vi "Current_Setting_1_7_26.vi"() -> ()   [LabVIEW 2025]
uses:
  <vilib>/addons/zeromq/zmq_socket.lvclass
  <vilib>/Waveform/DWDTOps.llb/DWDT Digital to Boolean Array.vi
  GV_TC1_M.vi
  <vilib>/DAQmx/read.llb/DAQmx Read (Analog DBL 1Chan 1Samp).vi
  <vilib>/DAQmx/read.llb/DAQmx Read (Analog 1D DBL NChan 1Samp).vi
  GV_TC1.vi
  <vilib>/addons/zeromq/zmq_context.lvclass
  <vilib>/addons/zeromq/socket_type.ctl
  <vilib>/addons/zeromq/zeromq.lvlib
  <vilib>/DAQmx/create/channels.llb/DAQmx Create Channel (AI-Voltage-Basic).vi
  <resource>/objmgr/daqmx.rc
  <vilib>/DAQmx/create/channels.llb/DAQmx Create Channel (AO-Voltage-Basic).vi
  <vilib>/DAQmx/write.llb/DAQmx Write (Analog DBL 1Chan 1Samp).vi
  GV_TC9_Mo.vi
panel:
  in  "stop":bool
  out "TC1_Command":dbl
  out "Waveform Chart":dbl(graph)
  out "Sign*10":dbl
  in  "Error_TC9":dbl
  in  "Inc/Dec":dbl
  in  "RF":tag
  in  "Others":tag
  out "error out":errorcluster
  out "double precision float":dbl
  out "Source 1":dbl
  out "Source 2":dbl
  out "Source 3":dbl
  out "Source 4":dbl
  out "Source 5":dbl
  out "Source 6":dbl
  out "Source 7":dbl
  out "Source 8":dbl
  out "Source 9":dbl
  out "Source 10":dbl
  out "Source 11":dbl
  out "Source 12":dbl
  out "Source 13":dbl
  out "Source 14":dbl
  out "value":dbl[](array[numeric])
  out "subarray":dbl[](array[numeric])
  out "Boolean array":bool[](array[boolean])
  out "TC 1":dbl
  out "TC 2":dbl
  out "TC 3":dbl
  out "TC 4":dbl
  out "TC 5":dbl
  out "TC 6":dbl
  out "TC 7":dbl
  out "TC 8":dbl
  out "going to Device 9":dbl
  out "going to Device 10":dbl
  out "going to Device 11":dbl
  out "going to Device 12":dbl
  out "going to Device 13":dbl
  out "going to Device 14":dbl
  in  "Numerator":dbl
  in  "Denominator":dbl
  in  "Inc/Dec 2":dbl
  in  "Error_Stop":dbl
  in  "Boolean":bool
  out "Array":dbl[](array[numeric])
  out "max value":i16
  out "Array[0]":dbl
  out "max value 2":i16
  out "Array 2":dbl[](array[numeric])
  in  "TP1":dbl
  in  "TP2":dbl
  in  "RF 2":dbl
  in  "Beam":dbl
  in  "Boolean 2":bool
  in  "Boolean 3":bool
  out "[0]":bool
  out "[1]":bool
  out "[2]":bool
  out "[3]":bool
  out "others":dbl[](array[numeric]) format="%0.2f"
  out "appended array":dbl[](array[numeric])
  out "x/y":dbl
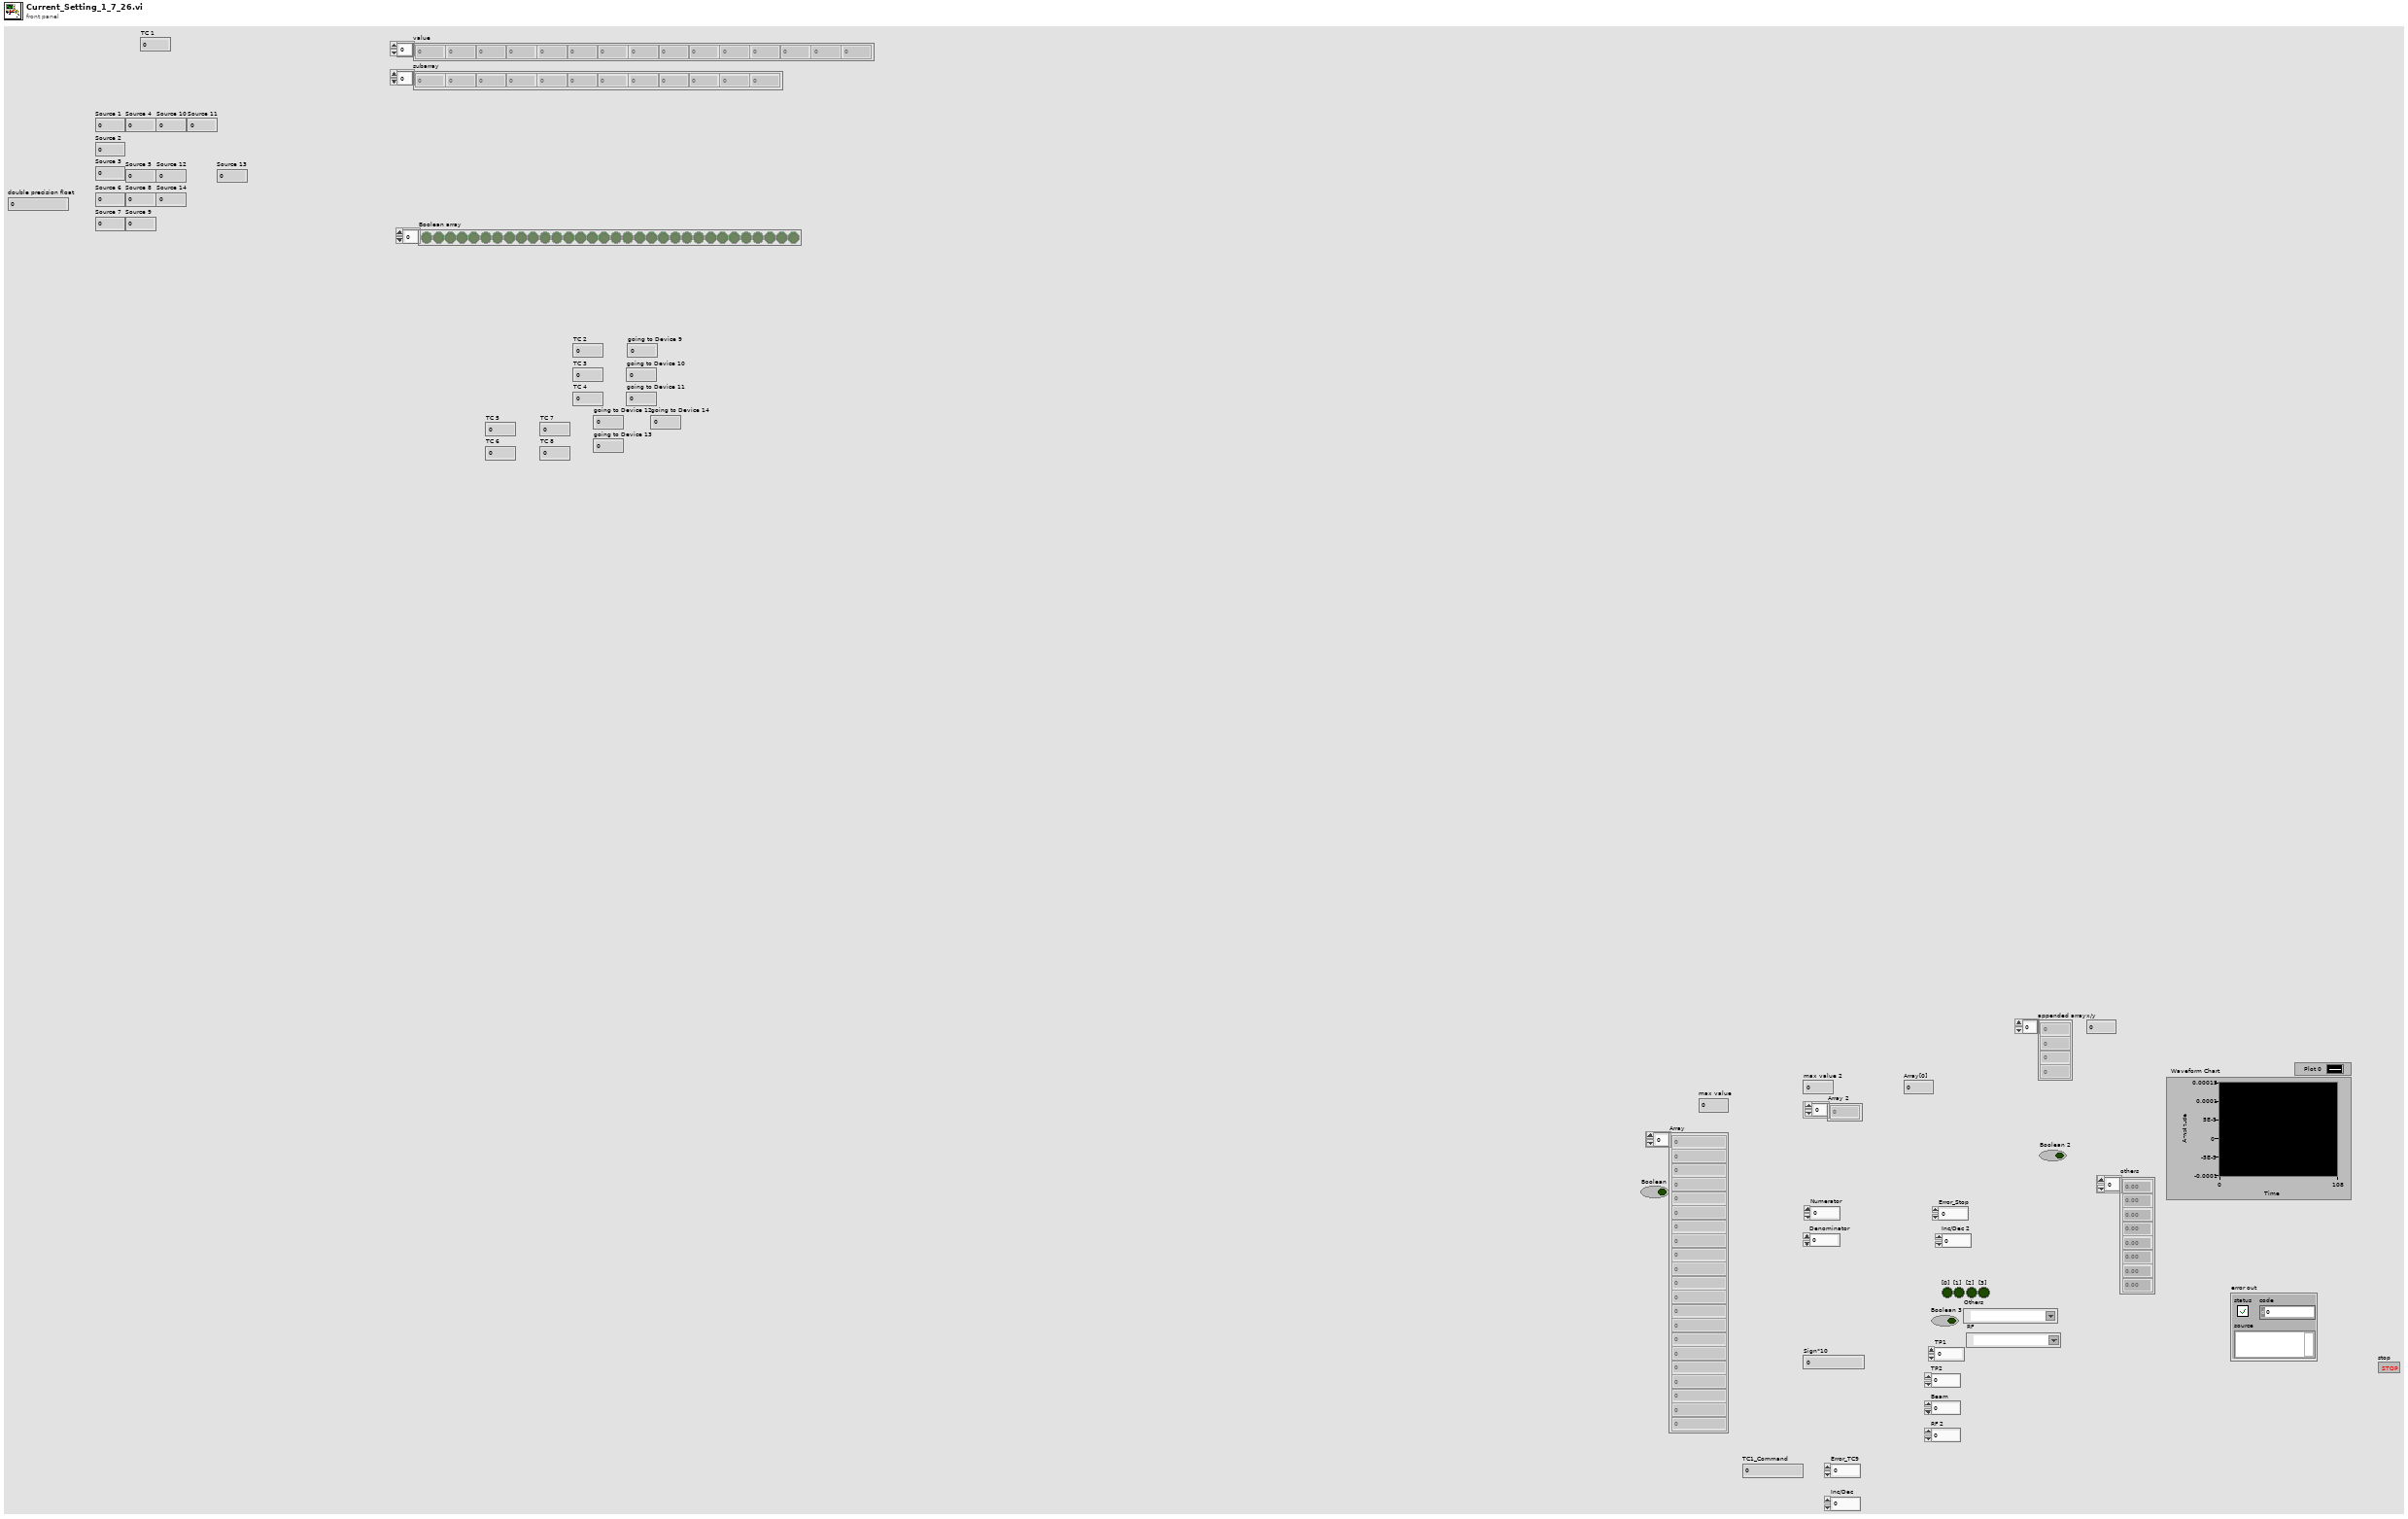
[diagram p1: front panel]
types:
  T1 = typedef "zeromq.lvlib/socket_type.ctl" = enum8{"ZMQ_PAIR", "ZMQ_PUB", "ZMQ_SUB", "ZMQ_REQ", "ZMQ_REP", "ZMQ_DEALER", "ZMQ_ROUTER", "ZMQ_PULL", "ZMQ_PUSH", "ZMQ_XPUB", "ZMQ_XSUB", "ZMQ_STREAM", "ZMQ_SERVER", "ZMQ_CLIENT", "ZMQ_RADIO", "ZMQ_DISH", "ZMQ_GATHER", "ZMQ_SCATTER", "ZMQ_DGRAM"}
  T2 = enum16{"big-endian, network order", "native, host order", "little-endian"}
  T3 = cluster{"[0]":bool, "[1]":bool, "[2]":bool, "[3]":bool, "[4]":bool, "[5]":bool, "[6]":bool, "[7]":bool, "[8]":bool}
  T4 = cluster{"[0]":dbl, "[1]":dbl, "[2]":dbl, "[3]":dbl, "[4]":dbl, "[5]":dbl, "[6]":dbl, "[7]":dbl}
  T5 = cluster{"Array[0]":dbl, "Array[1]":dbl, "Array[2]":dbl, "Array[3]":dbl, "Array[4]":dbl, "Array[5]":dbl, "Array[6]":dbl, "Array[7]":dbl}
  T6 = cluster{"[0]":digitalwaveform, "[1]":digitalwaveform, "[2]":digitalwaveform, "[3]":digitalwaveform, "[4]":digitalwaveform, "[5]":digitalwaveform, "[6]":digitalwaveform, "[7]":digitalwaveform, "[8]":digitalwaveform}
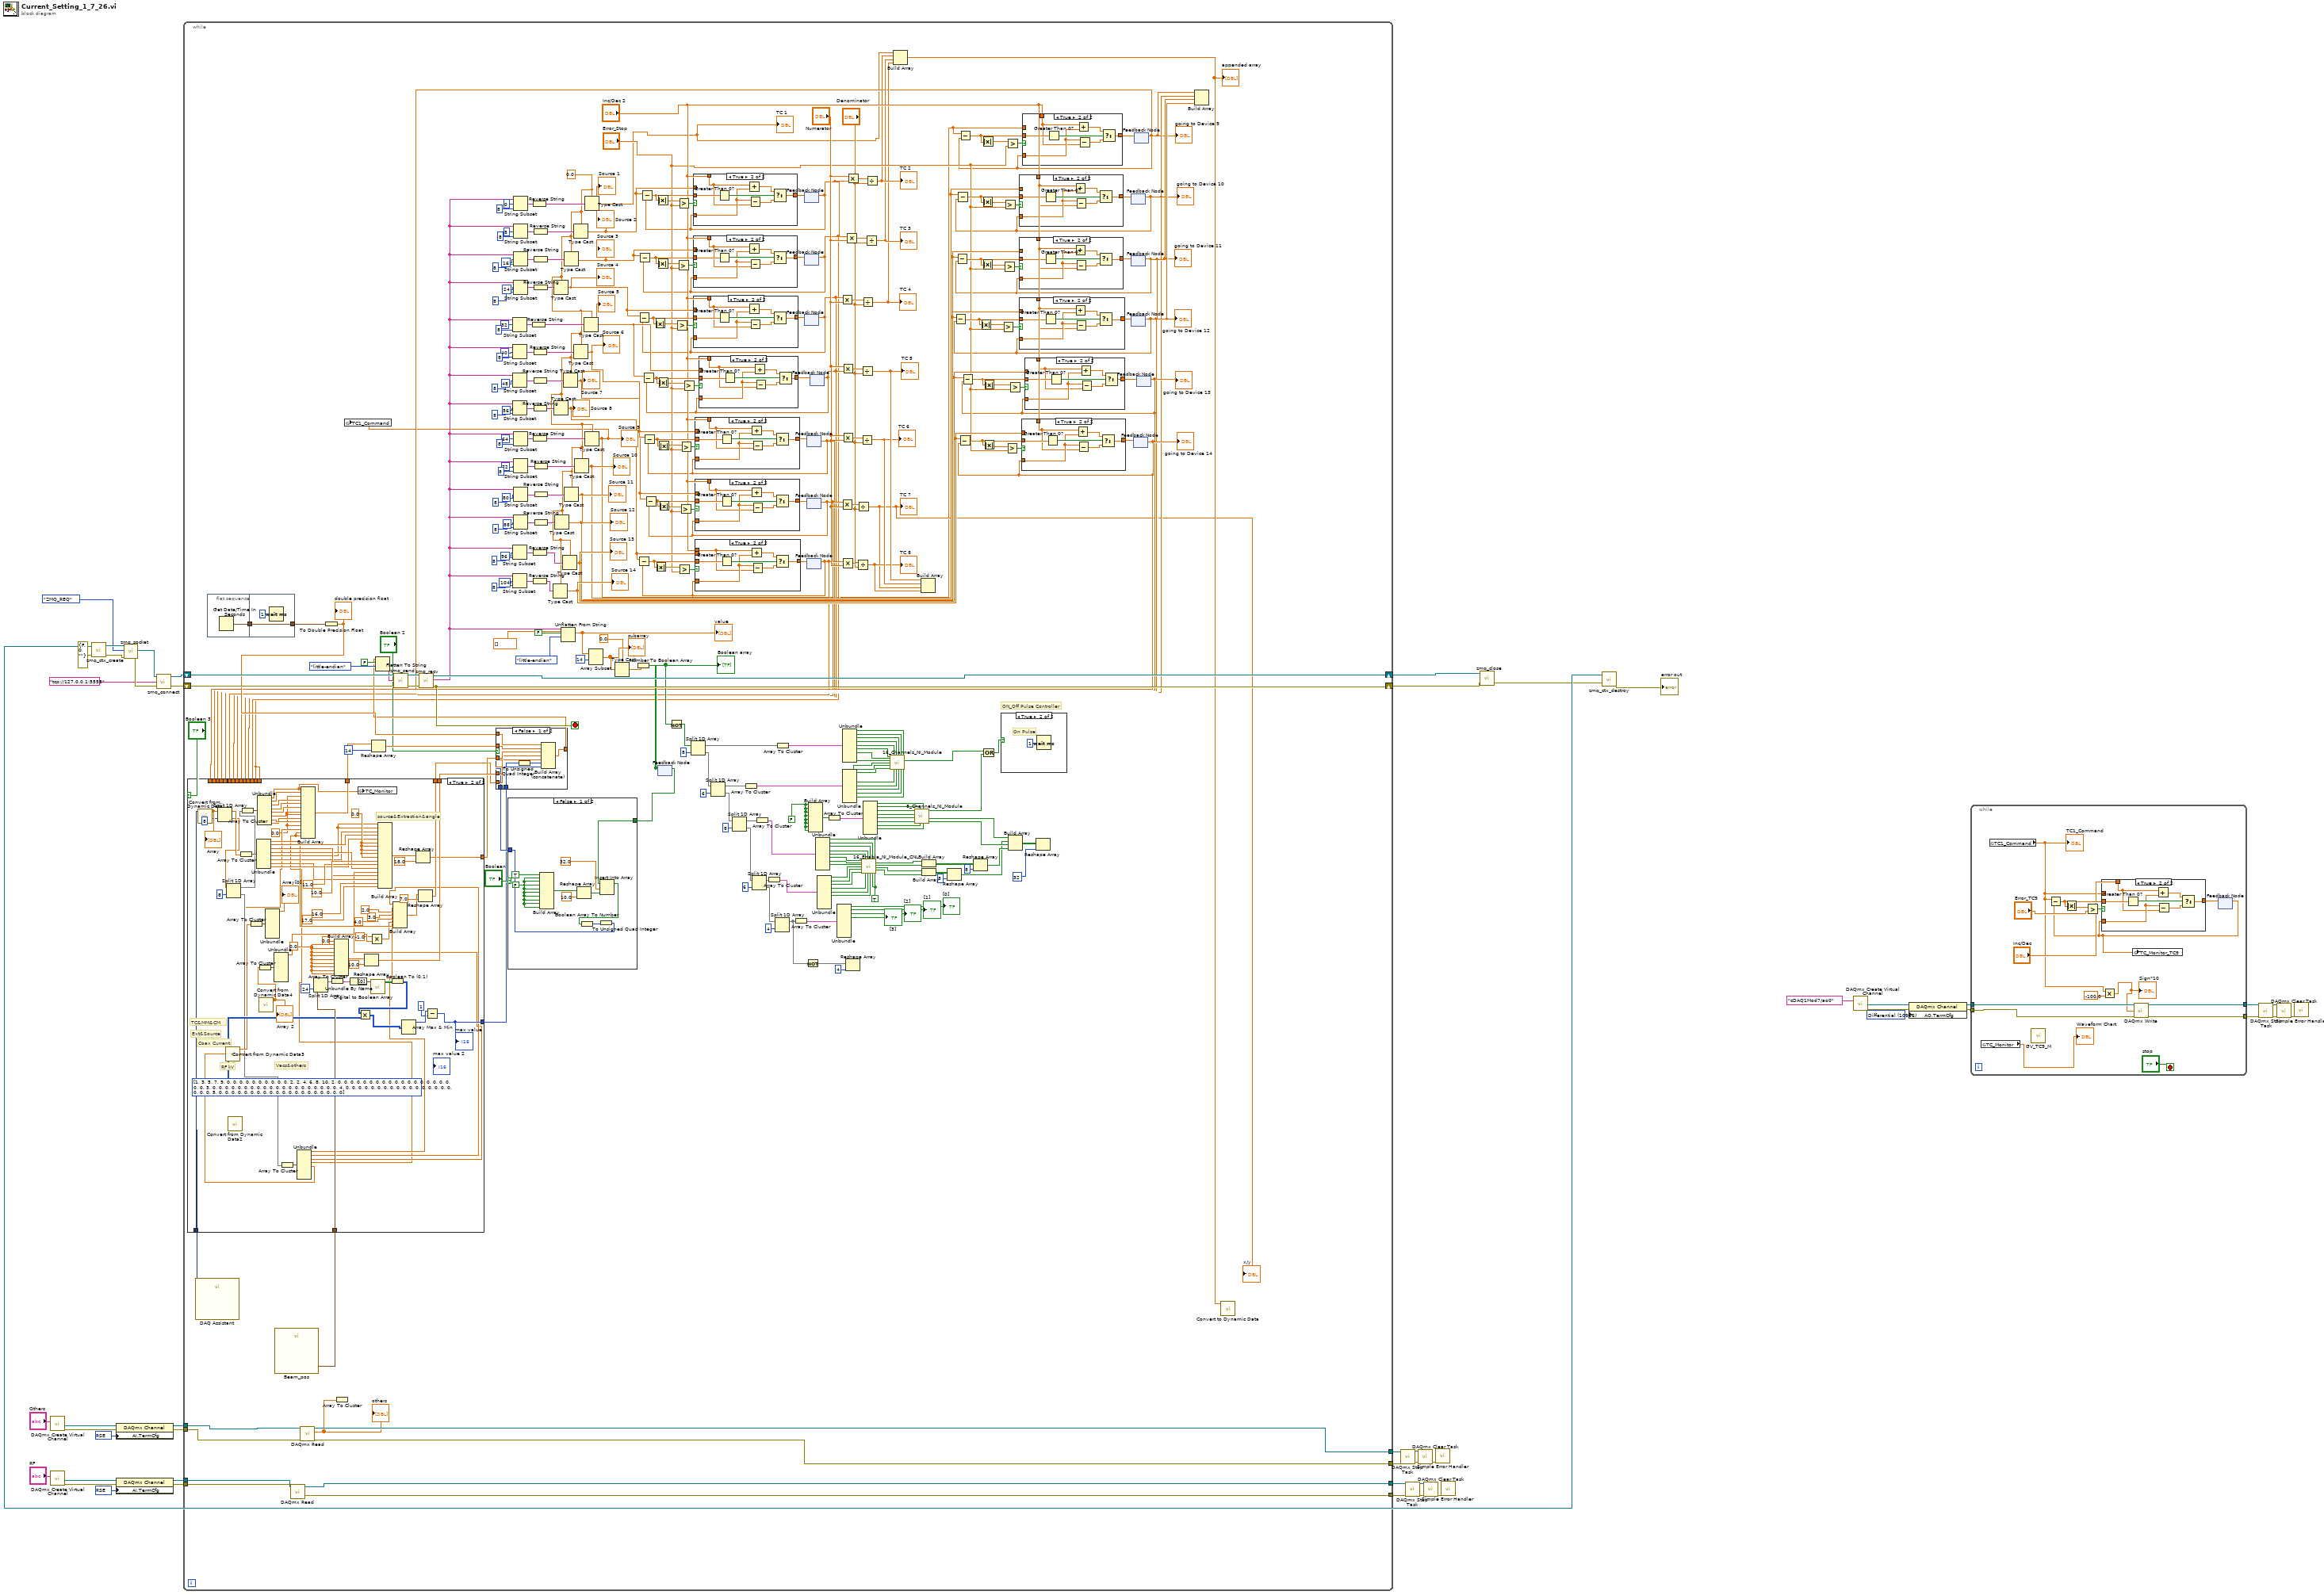
[diagram p0: block diagram]
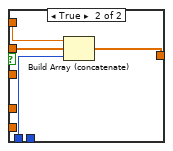
[diagram p3: hidden frame]
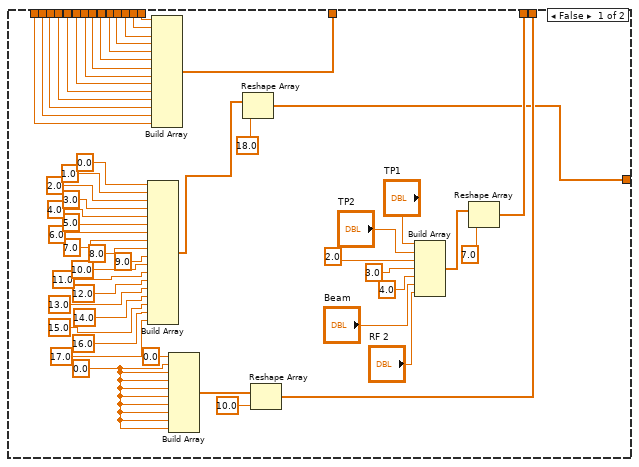
[diagram p4: hidden frame]
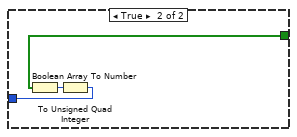
[diagram p5: hidden frame]
diagram:
  w8 = 10106 items=["RSE"=10083, "Differential"=10106, "Pseudodifferential"=12529] ("AO.TermCfg")
  w20 = 10083 items=["RSE"=10083, "Differential"=10106, "Pseudodifferential"=12529] ("AO.TermCfg")
  w31 = 10083 items=["RSE"=10083, "Differential"=10106, "Pseudodifferential"=12529] ("AO.TermCfg")
  n1 = call-poly <vilib>:"DAQmx Create Virtual Channel.vi"("physical channels"="Others") -> ("task out"=w32:refnum<k21>, "error out"=w33:errorcluster)  [unwired: 13 in]
  n2 = call-poly <vilib>:"DAQmx Create Virtual Channel.vi"("physical channels"="RF") -> ("task out"=w21:refnum<k21>, "error out"=w22:errorcluster)  [unwired: 13 in]
  n3 = call <vilib>:"zmq_ctx_create.vi"("error in"=errorcluster {"status"=FALSE, "code"=0, "source"=""}) -> ("error out"=w45:errorcluster, "context out"=w46:refnum<class "zmq_context.lvclass">)  [unwired: 3 in]
  n4 = property class="DAQmx Channel"(reference=w32, error in=w33, "AI.TermCfg"=w31) -> (reference out=w26:refnum<k21>, error out=w25:errorcluster)
  n5 = property class="DAQmx Channel"(reference=w21, error in=w22, "AI.TermCfg"=w20) -> (reference out=w18:refnum<k21>, error out=w17:errorcluster)
  n6 = call <vilib>:"zmq_socket.vi"("error in"=w45, "socket type"=socket_type."ZMQ_REQ", "context in"=w46) -> ("error out"=w43:errorcluster, "socket out"=w44:refnum<class "zmq_socket.lvclass">, "context out"=w38:refnum<class "zmq_context.lvclass">)  [unwired: 2 in]
  n7 = call <vilib>:"zmq_connect.vi"("error in"=w43, "endpoint"="tcp://127.0.0.1:5555", "socket in"=w44) -> ("error out"=w39:errorcluster, "socket out"=w40:refnum<class "zmq_socket.lvclass">)  [unwired: 1 in]
  n8 = while {
    shift-right: [w222] -> w35
    shift-left: w40 -> [w333]
    shift-right: [w221] -> w36
    shift-left: w39 -> [w332]
    tunnel: w26 -> [w79]
    tunnel: w25 -> [w78]
    tunnel: [w77] -> w24
    tunnel: [w76] -> w23
    tunnel: w18 -> [w75]
    tunnel: w17 -> [w74]
    tunnel: [w73] -> w13
    tunnel: [w72] -> w12
    stop <- w221 stop-if-true
    w112 = TRUE
    w115 = FALSE
    w261 = 0.0
    # "ON_Off Pulse Controller"
    n9 = call "DAQ Assistant"() -> ("data"=w54:dynamicdata)  [unwired: 16 in, 3 out]
    n10 = flat-sequence {
      tunnel: [w589] -> w328
      tunnel: [w591] -> w329
      tunnel: w328 -> [w591]
      frame #0 {
        n11 = Get Date/Time In Seconds() -> (seconds since 1Jan1904=w589:timestamp)
      }
      frame #1 {
        n12 = Wait (ms)(milliseconds to wait=u32 1) -> ()  [unwired: 1 out]
      }
    }
    n13 = call "Beam_pos"() -> ("data"=w55:digitalwaveform[])  [unwired: 16 in, 3 out]
    n14 = call-poly <vilib>:"DAQmx Read.vi"("task/channels in"=w75, "error in"=w74) -> ("task out"=w73:refnum<k21>, "error out"=w72:errorcluster)  [unwired: 11 in, 1 out]
    n15 = call-poly <vilib>:"DAQmx Read.vi"("task/channels in"=w79, "error in"=w78) -> ("task out"=w76:refnum<k21>, "data"=w71:dbl[], "error out"=w77:errorcluster)  [unwired: 11 in]
    "others" <- w71
    n16 = To Double Precision Float(number=w329) -> (double precision float=w99:dbl)
    "double precision float" <- w99
    n17 = Array To Cluster(array=w71) -> ()  [unwired: 1 out]
    n18 = feedback #1() -> (w102:bool[])  [unwired: 1 in]
    n19 = case shown="False" "Boolean" {
      tunnel: w102 -> [w476 w482]
      tunnel: [w473 w481] -> w100
      frame False {
        w479 = FALSE
        n20 = Build Array(TRUE, w479, w479, w479, w479, w479, w479, w479, w479, w479) -> (w478:bool[])
        n21 = Reshape Array(w478, 10.0) -> (w471:bool[])
        n22 = Insert Into Array(array=w476, index=32.0, new element=w471) -> (w474:bool[])
        n23 = Boolean Array To Number(Boolean array=w474) -> (number=w475:u32)
        n24 = To Unsigned Quad Integer(1:w475) -> (0:w473:u64)
      }
      frame True {
        n25 = Boolean Array To Number(Boolean array=w482) -> (number=w483:u32)
        n26 = To Unsigned Quad Integer(1:w483) -> (0:w481:u64)
      }
    }
    n27 = feedback #2() -> (w50:dbl)  [unwired: 1 in]
    n28 = feedback #3() -> (w59:dbl)  [unwired: 1 in]
    n29 = feedback #4() -> (w60:dbl)  [unwired: 1 in]
    n30 = feedback #5() -> (w62:dbl)  [unwired: 1 in]
    n31 = feedback #6() -> (w63:dbl)  [unwired: 1 in]
    n32 = feedback #7() -> (w64:dbl)  [unwired: 1 in]
    n33 = Build Array(w115, w115, w115, w115, w115, w115, w115, w115) -> (w113:bool[])
    n34 = feedback #8() -> (w61:dbl)  [unwired: 1 in]
    n35 = Array To Cluster(array=w113) -> (cluster=w114:T3)
    n36 = Multiply(x=w60, y="Numerator") -> (x*y=w216:dbl)
    n37 = Multiply(x=w63, y="Numerator") -> (x*y=w213:dbl)
    n38 = Multiply(x=w64, y="Numerator") -> (x*y=w212:dbl)
    n39 = Multiply(x="Numerator", y=w61) -> (x*y=w215:dbl)
    n40 = Multiply(x="Numerator", y=w62) -> (x*y=w214:dbl)
    n41 = Multiply(x=w59, y="Numerator") -> (x*y=w217:dbl)
    n42 = Multiply(x="Numerator", y=w50) -> (x*y=w218:dbl)
    n43 = Divide(x=w212, y="Denominator") -> (x/y=w103:dbl)
    "TC 8" <- w103
    n44 = Divide(x=w213, y="Denominator") -> (x/y=w51:dbl)
    "TC 7" <- w51
    "x/y" <- w51
    n45 = Divide(x=w214, y="Denominator") -> (x/y=w104:dbl)
    "TC 6" <- w104
    n46 = Divide(x=w215, y="Denominator") -> (x/y=w105:dbl)
    "TC 5" <- w105
    n47 = Divide(x=w216, y="Denominator") -> (x/y=w106:dbl)
    "TC 4" <- w106
    n48 = Unbundle(w114) -> ("[0]"=w149:bool, "[1]"=w148:bool, "[2]"=w147:bool, "[3]"=w146:bool, "[4]"=w145:bool, "[5]"=w144:bool, "[6]"=w143:bool, "[7]"=w142:bool)  [unwired: 1 out]
    n49 = Divide(x=w217, y="Denominator") -> (x/y=w107:dbl)
    "TC 3" <- w107
    n50 = Divide(x=w218, y="Denominator") -> (x/y=w108:dbl)
    "TC 2" <- w108
    n51 = call "8_Channels_NI_Module.vi"("Trigger 8"=w142, "Trigger"=w149, "Trigger 7"=w143, "Trigger 2"=w148, "Trigger 6"=w144, "Trigger 5"=w145, "Trigger 4"=w146, "Trigger 3"=w147) -> ("Off Array"=w140:bool[], "On Array"=w141:bool[], "Timing"=w111:bool)  [unwired: 1 in]
    n52 = Build Array(w105, w104, w51, w103) -> ()  [unwired: 1 out]
    n53 = feedback #9() -> (w66:dbl)  [unwired: 1 in]
    "going to Device 10" <- w66
    n54 = feedback #10() -> (w67:dbl)  [unwired: 1 in]
    "going to Device 11" <- w67
    n55 = feedback #11() -> (w68:dbl)  [unwired: 1 in]
    "going to Device 12" <- w68
    n56 = feedback #12() -> (w70:dbl)  [unwired: 1 in]
    "going to Device 14" <- w70
    n57 = feedback #13() -> (w65:dbl)  [unwired: 1 in]
    "going to Device 9" <- w65
    n58 = feedback #14() -> (w69:dbl)  [unwired: 1 in]
    "going to Device 13" <- w69
    n59 = case shown="True" "Boolean 3" {
      tunnel: [w372 w459] -> w94
      tunnel: [w366 w454] -> w93
      tunnel: [w369 w457] -> w92
      tunnel: w54 -> [_ w451]
      tunnel: w70 -> [w361 _]
      tunnel: w69 -> [w360 _]
      tunnel: w68 -> [w359 _]
      tunnel: w67 -> [w358 _]
      tunnel: w66 -> [w357 _]
      tunnel: w65 -> [w356 _]
      tunnel: w64 -> [w355 _]
      tunnel: w63 -> [w354 _]
      tunnel: w62 -> [w353 _]
      tunnel: w61 -> [w352 _]
      tunnel: w60 -> [w351 _]
      tunnel: w59 -> [w350 _]
      tunnel: w50 -> [w349 _]
      tunnel: w50 -> [w348 _]
      tunnel: [w347 w452] -> w57
      tunnel: w55 -> [_ w433]
      tunnel: [_ w421] -> w53
      frame False {
        w373 = 0.0 ("element")
        n60 = Build Array(0.0, 1.0, 2.0, 3.0, 4.0, 5.0, 6.0, 7.0, 8.0, 9.0, 10.0, 11.0, 12.0, 13.0, 14.0, 15.0, 16.0, 17.0) -> (w367:dbl[])
        n61 = Build Array(w348, w349, w350, w351, w352, w353, w354, w355, w356, w357, w358, w359, w360, w361) -> (w347:dbl[])
        n62 = Build Array(0.0 ("element"), w373, w373, w373, w373, w373, w373, w373, w373, w373) -> (w376:dbl[])
        n63 = Reshape Array(w367, 18.0) -> (w366:dbl[])
        n64 = Reshape Array(w376, 10.0) -> (w372:dbl[])
        n65 = Build Array("TP1", "TP2", 2.0, 3.0, 4.0, "Beam", "RF 2") -> (w370:dbl[])
        n66 = Reshape Array(w370, 7.0) -> (w369:dbl[])
      }
      frame True {
        w400 = 0.0
        w453 = 0.0
        w461 = 0.0 ("element")
        # "RF kV"
        # "Coax Current"
        # "Vacs&others"
        # "Ext&Source"
        # "TC&MM&CM"
        # "source&Extraction&angle"
        n67 = call "Convert from Dynamic Data"("Dynamic Data Type"=w451) -> ("Array"=w441:dbl[])  [unwired: 3 in]
        "Array" <- w441
        n68 = Split 1D Array(array=w441, index=8) -> (first subarray=w404:dbl[], second subarray=w403:dbl[])
        n69 = call "Convert from Dynamic Data3"() -> ("Array"=w423:dbl[])  [unwired: 4 in]
        n70 = Split 1D Array(array=w403, index=8) -> (first subarray=w402:dbl[], second subarray=w411:dbl[])
        n71 = call "Convert from Dynamic Data2"() -> ()  [unwired: 4 in, 1 out]
        n72 = Array To Cluster(array=w404) -> (cluster=w439:T4)
        n73 = Array To Cluster(array=w402) -> (cluster=w442:T4)
        n74 = Array To Cluster(array=w423) -> (cluster=w424:T5)
        n75 = Unbundle(w439) -> ("[0]"=w425:dbl, "[1]"=w438:dbl, "[2]"=w436:dbl, "[3]"=w435:dbl, "[4]"=w405:dbl, "[5]"=w406:dbl, "[6]"=w408:dbl, "[7]"=w437:dbl)
        n76 = Unbundle(w442) -> ("[0]"=w398:dbl, "[1]"=w450:dbl, "[2]"=w449:dbl, "[3]"=w448:dbl, "[4]"=w447:dbl, "[5]"=w446:dbl, "[6]"=w445:dbl, "[7]"=w444:dbl)
        n77 = call "Convert from Dynamic Data4"() -> ("Array"=w416:dbl[])  [unwired: 4 in]
        "Array 2" <- w416
        n78 = Array To Cluster(array=w416) -> (cluster=w417:T5)
        n79 = Unbundle(w424) -> ("Array[0]"=→"Array[0]":dbl)  [unwired: 7 out]
        n80 = Unbundle(w417) -> ("Array[0]"=w415:dbl)  [unwired: 7 out]
        n81 = Array To Cluster(array=w411) -> (cluster=w413:T4)
        n82 = Unbundle(w413) -> ("[0]"=w410:dbl, "[1]"=w409:dbl, "[2]"=w407:dbl, "[3]"=w399:dbl, "[4]"=w401:dbl)  [unwired: 3 out]
        n83 = Build Array(w398, w450, w400, w449, w448, w447, w446, w400, w444, w445, w400, w401, w399, w399) -> (w452:dbl[])
        n84 = Split 1D Array(array=w433, index=24) -> (first subarray=w430:digitalwaveform[])  [unwired: 1 out]
        n85 = Array To Cluster(array=w430) -> (cluster=w432:T6)
        n86 = Build Array(0.0 ("element"), w461, w461, w461, w461, w461, w461, w461, w461, w461) -> (w464:dbl[])
        n87 = Unbundle By Name(w432) -> ("[0]"=w431:digitalwaveform)
        n88 = global write "GV_TC1_M.vi" "TC_Monitor"(w398) -> ()
        n89 = Reshape Array(w464, 10.0) -> (w459:dbl[])
        n90 = Multiply(x=-1.0, y=w415) -> (x*y=w418:dbl)
        n91 = call-poly <vilib>:"Digital to Boolean Array.vi"("digital waveform"=w431) -> ("boolean array"=w429:bool[][])  [unwired: 9 in, 1 out]
        n92 = Build Array(w405, w405, w406, w438, w437, w453, w453, w453, w453, w453, 10.0, 11.0, w435, w407, w436, w408, 16.0, 17.0) -> (w455:dbl[])
        n93 = Boolean To (0,1)(Boolean=w429) -> (0, 1=w428:i16[][])
        n94 = Multiply(x=w428, y=i16[][] [[1, 3, 5, 7, 9, 0, 0, 0, 0, 0, 0, 0, 0, 0, 0, 2, 2, 4, 6, 8, 10], [2, 0, 0, 0, 0, 0, 0, 0, 0, 0, 0, 0, 0, 0, 0, 0, 0, 0, 0, 0, 0], [3, 0, 0, 0, 0, 0, 0, 0, 0, 0, 0, 0, 0, 0, 0, 0, 0, 0, 0, 0, 0], [4, 0, 0, 0, 0, 0, 0, 0, 0, 0, 0, 0, 0, 0, 0, 0, 0, 0, 0, 0, 0], [5, 0, 0, 0, 0, 0, 0, 0, 0, 0, 0, 0, 0, 0, 0, 0, 0, 0, 0, 0, 0]]) -> (x*y=w426:i16[][])
        n95 = Build Array(w409, w410, 2.0, 3.0, 4.0, w418, w425) -> (w458:dbl[])
        n96 = Array Max & Min(array=w426) -> (max value=w420:i16)  [unwired: 3 out]
        n97 = Reshape Array(w455, 18.0) -> (w454:dbl[])
        n98 = Reshape Array(w458, 7.0) -> (w457:dbl[])
        n99 = Subtract(x=w420, y=i16 1 ("x")) -> (x-y=w421:i16)
        "max value" <- w421
      }
    }
    n100 = Reshape Array(w57, 14 ("dimension size")) -> (w98:dbl[])
    n101 = case shown="False" "Boolean 2" {
      tunnel: w100 -> [w336 w346]
      tunnel: w99 -> [w342 w345]
      tunnel: w98 -> [w341 w344]
      tunnel: [w340 w343] -> w97
      tunnel: w94 -> [w338 _]
      tunnel: w93 -> [w339 _]
      tunnel: w92 -> [w337 _]
      tunnel: w53 -> [w334 _]
      frame False {
        n102 = To Unsigned Quad Integer(1:w334) -> (0:w335:u64)
        n103 = Build Array (concatenate)(w342, w341, w339, w338, w337, w335, w336) -> (w340:dbl[])
      }
      frame True {
        n104 = Build Array (concatenate)(w345, w344, w346) -> (w343:dbl[])
      }
    }
    n105 = Flatten To String(anything=w97, prepend array or string size? (T)=FALSE, byte order (0:big-endian, network order)=T2."little-endian") -> (data string=w220:string)  [unwired: 1 in, 2 out]
    n106 = call <vilib>:"zmq_send.vi"("error in"=w332, "data"=w220, "socket in"=w333) -> ("error out"=w330:errorcluster, "socket out"=w331:refnum<class "zmq_socket.lvclass">)  [unwired: 4 in]
    n107 = call <vilib>:"zmq_recv.vi"("error in"=w330, "socket in"=w331) -> ("error out"=w221:errorcluster, "data"=w219:string, "socket out"=w222:refnum<class "zmq_socket.lvclass">)  [unwired: 3 in, 2 out]
    n108 = String Subset(string=w219, offset (0)=96, length (rest)=8 ("length (rest)")) -> (substring=w273:string)
    n109 = String Subset(string=w219, offset (0)=104, length (rest)=8 ("length (rest)")) -> (substring=w271:string)
    n110 = String Subset(string=w219, offset (0)=32, length (rest)=8 ("length (rest)")) -> (substring=w305:string)
    n111 = String Subset(string=w219, offset (0)=40, length (rest)=8 ("length (rest)")) -> (substring=w303:string)
    n112 = String Subset(string=w219, offset (0)=48, length (rest)=8 ("length (rest)")) -> (substring=w297:string)
    n113 = String Subset(string=w219, offset (0)=56, length (rest)=8 ("length (rest)")) -> (substring=w295:string)
    n114 = String Subset(string=w219, offset (0)=0, length (rest)=8 ("length (rest)")) -> (substring=w321:string)
    n115 = String Subset(string=w219, offset (0)=8, length (rest)=8 ("length (rest)")) -> (substring=w319:string)
    n116 = String Subset(string=w219, offset (0)=16, length (rest)=8 ("length (rest)")) -> (substring=w313:string)
    n117 = String Subset(string=w219, offset (0)=24, length (rest)=8 ("length (rest)")) -> (substring=w311:string)
    n118 = String Subset(string=w219, offset (0)=64, length (rest)=8 ("length (rest)")) -> (substring=w289:string)
    n119 = String Subset(string=w219, offset (0)=72, length (rest)=8 ("length (rest)")) -> (substring=w287:string)
    n120 = String Subset(string=w219, offset (0)=80, length (rest)=8 ("length (rest)")) -> (substring=w281:string)
    n121 = String Subset(string=w219, offset (0)=88, length (rest)=8 ("length (rest)")) -> (substring=w279:string)
    n122 = Reverse String(1:w305) -> (0:w304:string)
    n123 = Reverse String(1:w321) -> (0:w320:string)
    n124 = Reverse String(1:w289) -> (0:w288:string)
    n125 = Reverse String(1:w273) -> (0:w272:string)
    n126 = Reverse String(1:w271) -> (0:w270:string)
    n127 = Reverse String(1:w303) -> (0:w302:string)
    n128 = Reverse String(1:w297) -> (0:w296:string)
    n129 = Reverse String(1:w295) -> (0:w294:string)
    n130 = Reverse String(1:w319) -> (0:w318:string)
    n131 = Reverse String(1:w313) -> (0:w312:string)
    n132 = Reverse String(1:w311) -> (0:w310:string)
    n133 = Reverse String(1:w287) -> (0:w286:string)
    n134 = Reverse String(1:w281) -> (0:w280:string)
    n135 = Reverse String(1:w279) -> (0:w278:string)
    n136 = Type Cast(type=w261, x=w270) -> (*(type *) &x=w227:dbl)
    "Source 14" <- w227
    n137 = Type Cast(type=w261, x=w294) -> (*(type *) &x=w240:dbl)
    "Source 8" <- w240
    n138 = Type Cast(type=w261, x=w310) -> (*(type *) &x=w252:dbl)
    "Source 4" <- w252
    n139 = Type Cast(type=w261, x=w278) -> (*(type *) &x=w225:dbl)
    "Source 12" <- w225
    n140 = Unflatten From String(type=dbl[] [], binary string=w219, data includes array or string size? (T)=FALSE, byte order (0:big-endian, network order)=T2."little-endian") -> (value=w266:dbl[])  [unwired: 1 in, 2 out]
    "value" <- w266
    n141 = Type Cast(type=w261, x=w272) -> (*(type *) &x=w226:dbl)
    "Source 13" <- w226
    n142 = Type Cast(type=w261, x=w296) -> (*(type *) &x=w241:dbl)
    "Source 7" <- w241
    n143 = Type Cast(type=w261, x=w312) -> (*(type *) &x=w253:dbl)
    "Source 3" <- w253
    n144 = Type Cast(type=w261, x=w280) -> (*(type *) &x=w224:dbl)
    "Source 11" <- w224
    n145 = Type Cast(type=w261, x=w302) -> (*(type *) &x=w242:dbl)
    "Source 6" <- w242
    n146 = Type Cast(type=w261, x=w318) -> (*(type *) &x=w254:dbl)
    "Source 2" <- w254
    n147 = Type Cast(type=w261, x=w286) -> (*(type *) &x=w223:dbl)
    "Source 10" <- w223
    n148 = Type Cast(type=w261, x=w304) -> (*(type *) &x=w243:dbl)
    "Source 5" <- w243
    n149 = Type Cast(type=w261, x=w320) -> (*(type *) &x=w49:dbl)
    "Source 1" <- w49
    "TC 1" <- w49
    n150 = Type Cast(type=w261, x=w288) -> (*(type *) &x=w48:dbl)
    "Source 9" <- w48
    n151 = global write "GV_TC1.vi" "TC1_Command"(w48) -> ()
    n152 = Array Subset(array=w266, index=14) -> (w264:dbl[])  [unwired: 1 in]
    "subarray" <- w264
    n153 = Type Cast(type=0.0, x=w264) -> (*(type *) &x=w262:dbl)
    n154 = Number To Boolean Array(number=w262) -> (Boolean array=w201:bool[])
    "Boolean array" <- w201
    n155 = Subtract(x=w240, y=w64) -> (x-y=w190:dbl)
    n156 = Subtract(x=w252, y=w60) -> (x-y=w195:dbl)
    n157 = Subtract(x=w253, y=w59) -> (x-y=w196:dbl)
    n158 = Subtract(x=w254, y=w50) -> (x-y=w199:dbl)
    n159 = Subtract(x=w243, y=w61) -> (x-y=w192:dbl)
    n160 = Subtract(x=w242, y=w62) -> (x-y=w187:dbl)
    n161 = Subtract(x=w241, y=w63) -> (x-y=w189:dbl)
    n162 = Absolute Value(x=w195) -> (abs(x)=w194:dbl)
    n163 = Absolute Value(x=w190) -> (abs(x)=w191:dbl)
    n164 = Absolute Value(x=w199) -> (abs(x)=w198:dbl)
    n165 = Absolute Value(x=w196) -> (abs(x)=w197:dbl)
    n166 = Absolute Value(x=w192) -> (abs(x)=w193:dbl)
    n167 = Absolute Value(x=w187) -> (abs(x)=w186:dbl)
    n168 = Absolute Value(x=w189) -> (abs(x)=w188:dbl)
    n169 = feedback-in #1(w201) -> ()
    n170 = Not(x=w201) -> (.not. x?=w200:bool[])
    n171 = Greater?(x=w194, y="Error_Stop") -> (0:w256:bool)
    n172 = Greater?(x=w197, y="Error_Stop") -> (0:w258:bool)
    n173 = Greater?(x=w198, y="Error_Stop") -> (0:w260:bool)
    n174 = Greater?(x=w191, y="Error_Stop") -> (0:w245:bool)
    n175 = Greater?(x=w188, y="Error_Stop") -> (0:w247:bool)
    n176 = Greater?(x=w186, y="Error_Stop") -> (0:w249:bool)
    n177 = Greater?(x=w193, y="Error_Stop") -> (0:w251:bool)
    n178 = Split 1D Array(array=w200, index=8) -> (first subarray=w210:bool[], second subarray=w209:bool[])
    n179 = case shown="True" w260 {
      tunnel: w199 -> [_ w588]
      tunnel: w50 -> [_ w586]
      tunnel: [w581 w583] -> w259
      tunnel: w254 -> [w581 _]
      tunnel: "Inc/Dec 2" -> [_ w582]
      frame False {
      }
      frame True {
        n180 = Greater Than 0?(x=w588) -> (x > 0?=w587:bool)
        n181 = Add(x=w582, y=w586) -> (x+y=w584:dbl)
        n182 = Subtract(x=w586, y=w582) -> (x-y=w585:dbl)
        n183 = Select(t=w584, s=w587, f=w585) -> (s? t:f=w583:dbl)
      }
    }
    n184 = case shown="True" w258 {
      tunnel: w196 -> [_ w580]
      tunnel: w59 -> [_ w578]
      tunnel: [w573 w575] -> w257
      tunnel: w253 -> [w573 _]
      tunnel: "Inc/Dec 2" -> [_ w574]
      frame False {
      }
      frame True {
        n185 = Greater Than 0?(x=w580) -> (x > 0?=w579:bool)
        n186 = Add(x=w574, y=w578) -> (x+y=w576:dbl)
        n187 = Subtract(x=w578, y=w574) -> (x-y=w577:dbl)
        n188 = Select(t=w576, s=w579, f=w577) -> (s? t:f=w575:dbl)
      }
    }
    n189 = case shown="True" w256 {
      tunnel: w195 -> [_ w572]
      tunnel: w60 -> [_ w570]
      tunnel: [w565 w567] -> w255
      tunnel: w252 -> [w565 _]
      tunnel: "Inc/Dec 2" -> [_ w566]
      frame False {
      }
      frame True {
        n190 = Greater Than 0?(x=w572) -> (x > 0?=w571:bool)
        n191 = Add(x=w566, y=w570) -> (x+y=w568:dbl)
        n192 = Subtract(x=w570, y=w566) -> (x-y=w569:dbl)
        n193 = Select(t=w568, s=w571, f=w569) -> (s? t:f=w567:dbl)
      }
    }
    n194 = case shown="True" w249 {
      tunnel: w187 -> [_ w556]
      tunnel: w62 -> [_ w554]
      tunnel: [w549 w551] -> w248
      tunnel: w242 -> [w549 _]
      tunnel: "Inc/Dec 2" -> [_ w550]
      frame False {
      }
      frame True {
        n195 = Greater Than 0?(x=w556) -> (x > 0?=w555:bool)
        n196 = Add(x=w550, y=w554) -> (x+y=w552:dbl)
        n197 = Subtract(x=w554, y=w550) -> (x-y=w553:dbl)
        n198 = Select(t=w552, s=w555, f=w553) -> (s? t:f=w551:dbl)
      }
    }
    n199 = case shown="True" w247 {
      tunnel: w189 -> [_ w548]
      tunnel: w63 -> [_ w546]
      tunnel: [w541 w543] -> w246
      tunnel: w241 -> [w541 _]
      tunnel: "Inc/Dec 2" -> [_ w542]
      frame False {
      }
      frame True {
        n200 = Greater Than 0?(x=w548) -> (x > 0?=w547:bool)
        n201 = Add(x=w542, y=w546) -> (x+y=w544:dbl)
        n202 = Subtract(x=w546, y=w542) -> (x-y=w545:dbl)
        n203 = Select(t=w544, s=w547, f=w545) -> (s? t:f=w543:dbl)
      }
    }
    n204 = case shown="True" w245 {
      tunnel: w190 -> [_ w540]
      tunnel: w64 -> [_ w538]
      tunnel: [w533 w535] -> w244
      tunnel: w240 -> [w533 _]
      tunnel: "Inc/Dec 2" -> [_ w534]
      frame False {
      }
      frame True {
        n205 = Greater Than 0?(x=w540) -> (x > 0?=w539:bool)
        n206 = Add(x=w534, y=w538) -> (x+y=w536:dbl)
        n207 = Subtract(x=w538, y=w534) -> (x-y=w537:dbl)
        n208 = Select(t=w536, s=w539, f=w537) -> (s? t:f=w535:dbl)
      }
    }
    n209 = case shown="True" w251 {
      tunnel: w192 -> [_ w564]
      tunnel: w61 -> [_ w562]
      tunnel: [w557 w559] -> w250
      tunnel: w243 -> [w557 _]
      tunnel: "Inc/Dec 2" -> [_ w558]
      frame False {
      }
      frame True {
        n210 = Greater Than 0?(x=w564) -> (x > 0?=w563:bool)
        n211 = Add(x=w558, y=w562) -> (x+y=w560:dbl)
        n212 = Subtract(x=w562, y=w558) -> (x-y=w561:dbl)
        n213 = Select(t=w560, s=w563, f=w561) -> (s? t:f=w559:dbl)
      }
    }
    n214 = Split 1D Array(array=w209, index=6) -> (first subarray=w207:bool[], second subarray=w205:bool[])
    n215 = Split 1D Array(array=w205, index=8) -> (first subarray=w204:bool[], second subarray=w202:bool[])
    n216 = Array To Cluster(array=w207) -> (cluster=w150:T3)
    n217 = Split 1D Array(array=w202, index=6) -> (first subarray=w203:bool[], second subarray=w89:bool[])
    n218 = Array To Cluster(array=w204) -> (cluster=w109:T3)
    n219 = Array To Cluster(array=w203) -> (cluster=w110:T3)
    n220 = Array To Cluster(array=w210) -> (cluster=w153:T3)
    n221 = Split 1D Array(array=w89, index=4) -> (first subarray=w81:bool[])  [unwired: 1 out]
    n222 = Array To Cluster(array=w81) -> (cluster=w88:T3)
    n223 = feedback-in #2(w259) -> ()
    n224 = feedback-in #3(w257) -> ()
    n225 = feedback-in #4(w255) -> ()
    n226 = Not(x=w81) -> (.not. x?=w80:bool[])
    n227 = feedback-in #5(w248) -> ()
    n228 = feedback-in #6(w246) -> ()
    n229 = feedback-in #7(w244) -> ()
    n230 = feedback-in #8(w250) -> ()
    n231 = Unbundle(w109) -> ("[0]"=w139:bool, "[1]"=w138:bool, "[2]"=w137:bool, "[3]"=w136:bool, "[4]"=w135:bool, "[5]"=w134:bool, "[6]"=w133:bool, "[7]"=w132:bool)  [unwired: 1 out]
    n232 = Unbundle(w110) -> ("[0]"=w127:bool, "[1]"=w126:bool, "[2]"=w125:bool, "[3]"=w124:bool, "[4]"=w91:bool, "[5]"=w90:bool)  [unwired: 3 out]
    n233 = Unbundle(w88) -> ("[0]"=→"[0]":bool, "[1]"=→"[1]":bool, "[2]"=→"[2]":bool, "[3]"=→"[3]":bool)  [unwired: 5 out]
    n234 = Unbundle(w153) -> ("[0]"=w154:bool, "[1]"=w169:bool, "[2]"=w168:bool, "[3]"=w167:bool, "[4]"=w166:bool, "[5]"=w165:bool, "[6]"=w164:bool, "[7]"=w163:bool)  [unwired: 1 out]
    n235 = Unbundle(w150) -> ("[0]"=w162:bool, "[1]"=w161:bool, "[2]"=w160:bool, "[3]"=w159:bool, "[4]"=w158:bool, "[5]"=w157:bool, "[6]"=w156:bool, "[7]"=w155:bool)  [unwired: 1 out]
    n236 = Reshape Array(w80, 4 ("dimension size")) -> ()  [unwired: 1 out]
    n237 = call "16_Enable_NI_Module_CNL.vi"("Enable 6"=w134, "Enable 7"=w133, "Enable 8"=w132, "Enable 9"=w127, "Enable 10"=w126, "Enable 11"=w125, "Enable 5"=w135, "Enable 12"=w124, "Enable 4"=w136, "Enable 13"=w91, "Enable 3"=w137, "Enable 14"=w90, "Enable 2"=w138, "Enable 15"=w112, "Enable 1"=w139, "Enable16"=w112) -> ("9_11_13_15"=w131:bool[], "1_3_5_7"=w130:bool[], "10_12_14_16"=w122:bool[], "2_4_6_8"=w121:bool[])
    n238 = call "16_Channels_NI_Module.vi"("Trigger 6"=w165, "Trigger 7"=w164, "Trigger 8"=w163, "Trigger 9"=w162, "Trigger 10"=w161, "Trigger 11"=w160, "Trigger 5"=w166, "Trigger 12"=w159, "Trigger 4"=w167, "Trigger 13"=w158, "Trigger 3"=w168, "Trigger 14"=w157, "Trigger 2"=w169, "Trigger 15"=w156, "Trigger"=w154, "Trigger 16"=w155) -> ("Timing"=w151:bool)  [unwired: 2 in, 1 out]
    n239 = Build Array(w49, w108, w107, w106) -> (w52:dbl[])
    "appended array" <- w52
    n240 = Build Array(w131, w130) -> (w128:bool[][])
    n241 = Build Array(w122, w121) -> (w120:bool[][])
    n242 = Reshape Array(w120, 8 ("dimension size")) -> (w116:bool[])
    n243 = Subtract(x=w225, y=w68) -> (x-y=w178:dbl)
    n244 = Subtract(x=w224, y=w67) -> (x-y=w180:dbl)
    n245 = Subtract(x=w223, y=w66) -> (x-y=w182:dbl)
    n246 = Subtract(x=w227, y=w70) -> (x-y=w174:dbl)
    n247 = Subtract(x=w48, y=w65) -> (x-y=w184:dbl)
    n248 = Subtract(x=w226, y=w69) -> (x-y=w176:dbl)
    n249 = Reshape Array(w128, 8 ("dimension size")) -> (w117:bool[])
    n250 = Absolute Value(x=w178) -> (abs(x)=w179:dbl)
    n251 = Absolute Value(x=w182) -> (abs(x)=w183:dbl)
    n252 = Absolute Value(x=w180) -> (abs(x)=w181:dbl)
    n253 = Absolute Value(x=w184) -> (abs(x)=w185:dbl)
    n254 = Absolute Value(x=w176) -> (abs(x)=w177:dbl)
    n255 = Absolute Value(x=w174) -> (abs(x)=w175:dbl)
    n256 = Compound Arithmetic op=OR(w151, w111) -> (w152:bool)
    n257 = Greater?(x=w179, y="Error_Stop") -> (0:w233:bool)
    n258 = case shown="True" w152 {
      frame False {
      }
      frame True {
        # "On Pulse"
        n259 = Wait (ms)(milliseconds to wait=u32 1) -> ()  [unwired: 1 out]
      }
    }
    n260 = Greater?(x=w181, y="Error_Stop") -> (0:w235:bool)
    n261 = Greater?(x=w183, y="Error_Stop") -> (0:w237:bool)
    n262 = Greater?(x=w175, y="Error_Stop") -> (0:w229:bool)
    n263 = Greater?(x=w185, y="Error_Stop") -> (0:w239:bool)
    n264 = Greater?(x=w177, y="Error_Stop") -> (0:w231:bool)
    n265 = Build Array(w141, w116, w140, w117) -> (w119:bool[][])
    n266 = case shown="True" w237 {
      tunnel: w182 -> [_ w524]
      tunnel: w66 -> [_ w522]
      tunnel: [w517 w519] -> w236
      tunnel: w223 -> [w517 _]
      tunnel: "Inc/Dec 2" -> [_ w518]
      frame False {
      }
      frame True {
        n267 = Greater Than 0?(x=w524) -> (x > 0?=w523:bool)
        n268 = Add(x=w518, y=w522) -> (x+y=w520:dbl)
        n269 = Subtract(x=w522, y=w518) -> (x-y=w521:dbl)
        n270 = Select(t=w520, s=w523, f=w521) -> (s? t:f=w519:dbl)
      }
    }
    n271 = case shown="True" w235 {
      tunnel: w180 -> [_ w516]
      tunnel: w67 -> [_ w514]
      tunnel: [w509 w511] -> w234
      tunnel: w224 -> [w509 _]
      tunnel: "Inc/Dec 2" -> [_ w510]
      frame False {
      }
      frame True {
        n272 = Greater Than 0?(x=w516) -> (x > 0?=w515:bool)
        n273 = Add(x=w510, y=w514) -> (x+y=w512:dbl)
        n274 = Subtract(x=w514, y=w510) -> (x-y=w513:dbl)
        n275 = Select(t=w512, s=w515, f=w513) -> (s? t:f=w511:dbl)
      }
    }
    n276 = case shown="True" w233 {
      tunnel: w178 -> [_ w508]
      tunnel: w68 -> [_ w506]
      tunnel: [w501 w503] -> w232
      tunnel: w225 -> [w501 _]
      tunnel: "Inc/Dec 2" -> [_ w502]
      frame False {
      }
      frame True {
        n277 = Greater Than 0?(x=w508) -> (x > 0?=w507:bool)
        n278 = Add(x=w502, y=w506) -> (x+y=w504:dbl)
        n279 = Subtract(x=w506, y=w502) -> (x-y=w505:dbl)
        n280 = Select(t=w504, s=w507, f=w505) -> (s? t:f=w503:dbl)
      }
    }
    n281 = case shown="True" w229 {
      tunnel: w174 -> [_ w492]
      tunnel: w70 -> [_ w490]
      tunnel: [w485 w487] -> w228
      tunnel: w227 -> [w485 _]
      tunnel: "Inc/Dec 2" -> [_ w486]
      frame False {
      }
      frame True {
        n282 = Greater Than 0?(x=w492) -> (x > 0?=w491:bool)
        n283 = Add(x=w486, y=w490) -> (x+y=w488:dbl)
        n284 = Subtract(x=w490, y=w486) -> (x-y=w489:dbl)
        n285 = Select(t=w488, s=w491, f=w489) -> (s? t:f=w487:dbl)
      }
    }
    n286 = case shown="True" w239 {
      tunnel: w184 -> [_ w532]
      tunnel: w65 -> [_ w530]
      tunnel: [w525 w527] -> w238
      tunnel: w48 -> [w525 _]
      tunnel: "Inc/Dec 2" -> [_ w526]
      frame False {
      }
      frame True {
        n287 = Greater Than 0?(x=w532) -> (x > 0?=w531:bool)
        n288 = Add(x=w526, y=w530) -> (x+y=w528:dbl)
        n289 = Subtract(x=w530, y=w526) -> (x-y=w529:dbl)
        n290 = Select(t=w528, s=w531, f=w529) -> (s? t:f=w527:dbl)
      }
    }
    n291 = case shown="True" w231 {
      tunnel: w176 -> [_ w500]
      tunnel: w69 -> [_ w498]
      tunnel: [w493 w495] -> w230
      tunnel: w226 -> [w493 _]
      tunnel: "Inc/Dec 2" -> [_ w494]
      frame False {
      }
      frame True {
        n292 = Greater Than 0?(x=w500) -> (x > 0?=w499:bool)
        n293 = Add(x=w494, y=w498) -> (x+y=w496:dbl)
        n294 = Subtract(x=w498, y=w494) -> (x-y=w497:dbl)
        n295 = Select(t=w496, s=w499, f=w497) -> (s? t:f=w495:dbl)
      }
    }
    n296 = Reshape Array(w119, 32 ("dimension size")) -> ()  [unwired: 1 out]
    n297 = feedback-in #9(w236) -> ()
    n298 = feedback-in #10(w234) -> ()
    n299 = feedback-in #11(w232) -> ()
    n300 = feedback-in #12(w228) -> ()
    n301 = feedback-in #13(w238) -> ()
    n302 = feedback-in #14(w230) -> ()
    n303 = Build Array(w65, w66, w67, w68) -> ()  [unwired: 1 out]
    n304 = call "Convert to Dynamic Data"("Array"=w52) -> ()  [unwired: 3 in, 1 out]
  }
  n305 = call <vilib>:"DAQmx Stop Task.vi"("task/channels in"=w23, "error in"=w24) -> ("task out"=w29:refnum<k21>, "error out"=w28:errorcluster)  [unwired: 12 in]
  n306 = call <vilib>:"DAQmx Stop Task.vi"("task/channels in"=w13, "error in"=w12) -> ("task out"=w16:refnum<k21>, "error out"=w15:errorcluster)  [unwired: 12 in]
  n307 = call <vilib>:"DAQmx Clear Task.vi"("task in"=w29, "error in"=w28) -> ("error out"=w27:errorcluster)  [unwired: 13 in]
  n308 = call <vilib>:"DAQmx Clear Task.vi"("task in"=w16, "error in"=w15) -> ("error out"=w14:errorcluster)  [unwired: 13 in]
  n309 = call <vilib>:"Simple Error Handler.vi"("error in (no error)"=w27) -> ()  [unwired: 4 in, 5 out]
  n310 = call <vilib>:"Simple Error Handler.vi"("error in (no error)"=w14) -> ()  [unwired: 4 in, 5 out]
  n311 = call <vilib>:"zmq_close.vi"("error in"=w36, "socket"=w35) -> ("error out"=w37:errorcluster)  [unwired: 3 in]
  n312 = call <vilib>:"zmq_ctx_destroy.vi"("error in"=w37, "context in"=w38) -> ("error out"=→"error out":errorcluster)  [unwired: 3 in]
  n313 = call-poly <vilib>:"DAQmx Create Virtual Channel.vi"("physical channels"=tag "cDAQ1Mod7/ao0") -> ("task out"=w10:refnum<k21>, "error out"=w11:errorcluster)  [unwired: 13 in]
  n314 = property class="DAQmx Channel"(reference=w10, error in=w11, "AO.TermCfg"=w8) -> (reference out=w4:refnum<k21>, error out=w3:errorcluster)
  n315 = while {
    tunnel: w4 -> [w607]
    tunnel: w3 -> [w606]
    tunnel: [w605] -> w2
    tunnel: [w604] -> w1
    stop <- "stop" stop-if-true
    n316 = global read "GV_TC1_M.vi" "TC_Monitor"() -> (→"Waveform Chart":dbl)
    n317 = global read "GV_TC1.vi" "TC1_Command"() -> (w592:dbl)
    "TC1_Command" <- w592
    n318 = call "GV_TC9_M.vi"() -> ()  [unwired: 12 in]
    n319 = Multiply(x=w592, y=-100.0) -> (x*y=w601:dbl)
    "Sign*10" <- w601
    n320 = call-poly <vilib>:"DAQmx Write.vi"("task/channels in"=w607, "data"=w601, "error in"=w606) -> ("task out"=w605:refnum<k21>, "error out"=w604:errorcluster)  [unwired: 10 in, 1 out]
    n321 = feedback #15() -> (w594:dbl)  [unwired: 1 in]
    n322 = Subtract(x=w592, y=w594) -> (x-y=w599:dbl)
    n323 = Absolute Value(x=w599) -> (abs(x)=w600:dbl)
    n324 = Greater?(x=w600, y="Error_TC9") -> (0:w598:bool)
    n325 = case shown="True" w598 {
      tunnel: w599 -> [_ w615]
      tunnel: w594 -> [_ w613]
      tunnel: [w608 w610] -> w597
      tunnel: w592 -> [w608 _]
      tunnel: "Inc/Dec" -> [_ w609]
      frame False {
      }
      frame True {
        n326 = Greater Than 0?(x=w615) -> (x > 0?=w614:bool)
        n327 = Add(x=w609, y=w613) -> (x+y=w611:dbl)
        n328 = Subtract(x=w613, y=w609) -> (x-y=w612:dbl)
        n329 = Select(t=w611, s=w614, f=w612) -> (s? t:f=w610:dbl)
      }
    }
    n330 = global write "GV_TC9_Mo.vi" "TC_Monitor_TC9"(w594) -> ()
    n331 = feedback-in #15(w597) -> ()
  }
  n332 = call <vilib>:"DAQmx Stop Task.vi"("task/channels in"=w2, "error in"=w1) -> ("task out"=w7:refnum<k21>, "error out"=w6:errorcluster)  [unwired: 12 in]
  n333 = call <vilib>:"DAQmx Clear Task.vi"("task in"=w7, "error in"=w6) -> ("error out"=w5:errorcluster)  [unwired: 13 in]
  n334 = call <vilib>:"Simple Error Handler.vi"("error in (no error)"=w5) -> ()  [unwired: 4 in, 5 out]
